vi "P-612 Stage Engine.vi"(0 "Unique Notifier Name":string, 11 "COM Port":string[](array[string])) -> ()   [LabVIEW 2016]
uses:
  Stages Controls/Stage Status.ctl
  Stages Controls/Stage XY Control.ctl
  Stages Controls/Stage Notifier Element.ctl
  Stages Controls/Stage Actions.ctl
panel:
  in  "XY Control":T1={"Left"=FALSE, "Right"=FALSE, "Up"=FALSE, "Down"=FALSE, "Home"=FALSE, "StageStep"=enum."1", "Y"=0.0, "X"=0.0}
  in  "ReInitialize":bool
  in  "Error":bool
  out "Status":T2
  in  "QUIT":bool
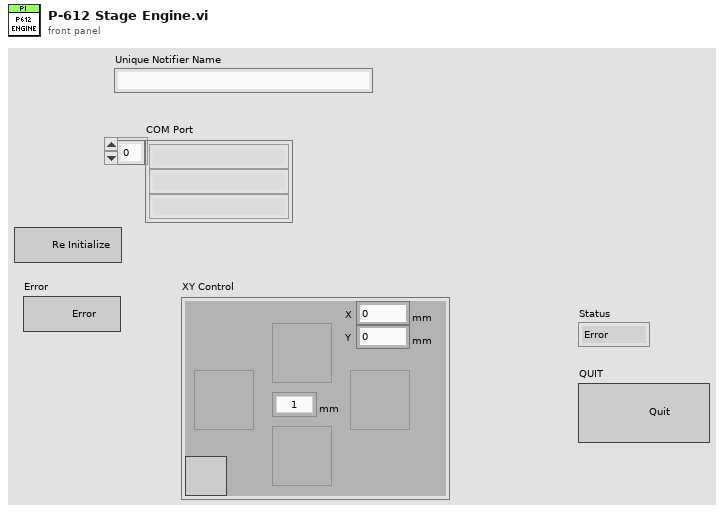
[diagram p1: front panel]
types:
  T1 = typedef "Stage XY Control.ctl" = cluster{"Left":bool, "Right":bool, "Up":bool, "Down":bool, "Home":bool, "StageStep":enum16{"0.01", "0.02", "0.05", "0.1", "0.5", "1", "2", "5", "10", "20", "50", "100", "500", "1000", "2000", "5000"}, "Y":dbl, "X":dbl}
  T2 = typedef "Stage Status.ctl" = enum16{"Error", "Abort", "Busy", "On Target"}
  T3 = typedef "Stage Actions.ctl" = enum16{"Get Position", "MVR", "MOVE", "HALT", "ONTARGET", "ERROR", "REFERENCE", "INIT", "VELOCITY", "STATUS", "EXIT", "HOME", "ZEROPOS", "NANOPOS", "ANALOG", "QUIT"}
  T4 = typedef "Stage Notifier Element.ctl" = cluster{"Action":T3, "Axis":bool[], "Setpoint":dbl[], "Velocity":dbl, "Cmd Recvd?":bool, "Position":dbl[], "Status":T2, "Misc":variant}
  T5 = cluster{"Left":bool, "Right":bool, "Up":bool, "Down":bool, "Home":bool, "StageStep":bool, "Y":bool, "X":bool}
  T6 = enum16{"0.01", "0.02", "0.05", "0.1", "0.5", "1", "2", "5", "10", "20", "50", "100", "500", "1000", "2000", "5000"}
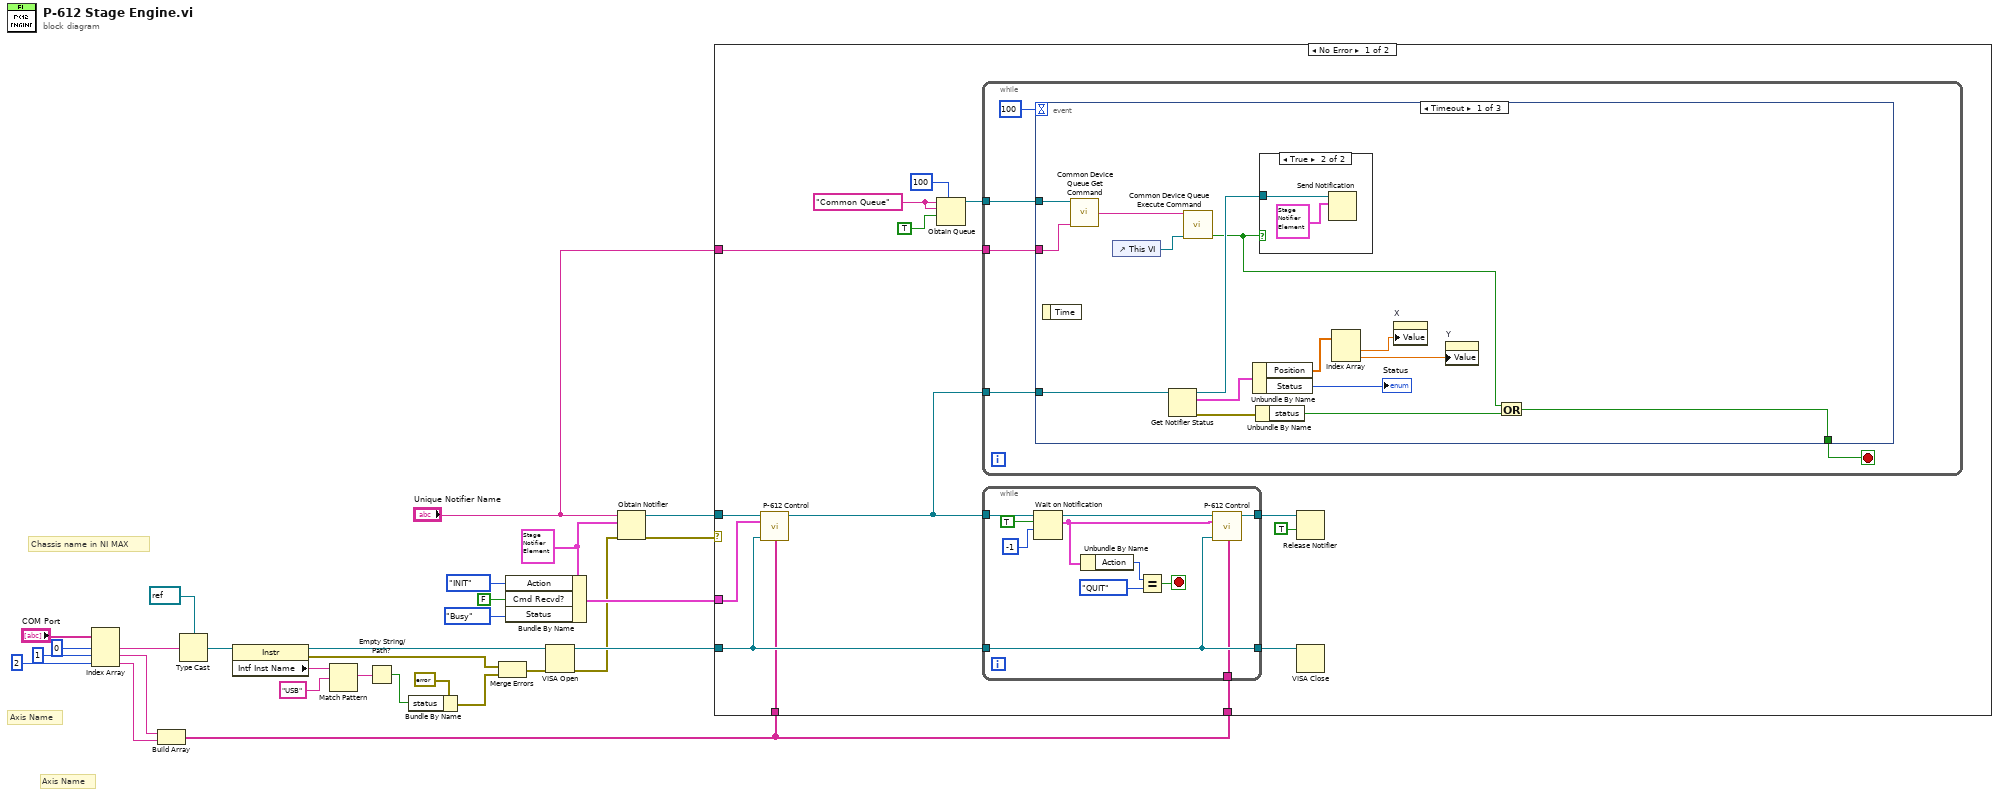
[diagram p0: block diagram]
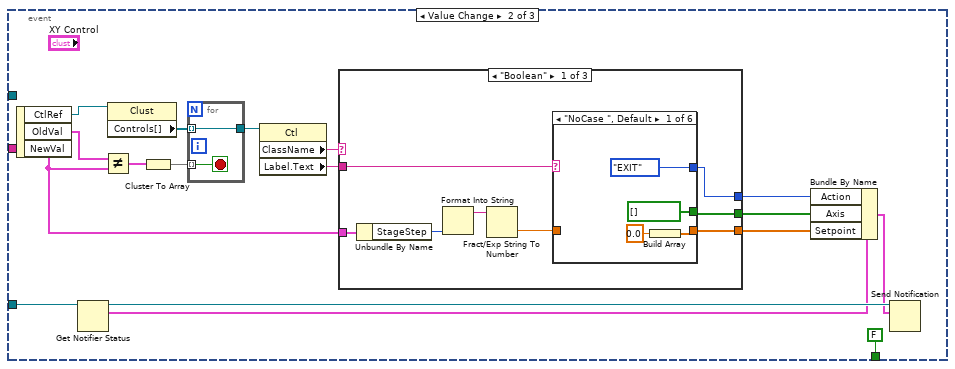
[diagram p3: hidden frame]
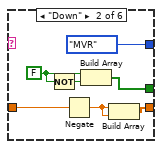
[diagram p4: hidden frame]
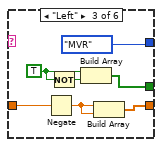
[diagram p5: hidden frame]
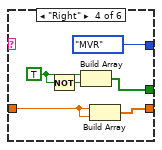
[diagram p6: hidden frame]
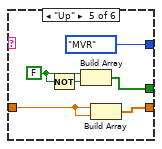
[diagram p7: hidden frame]
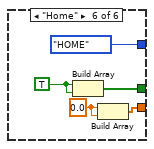
[diagram p8: hidden frame]
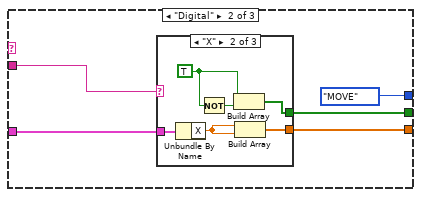
[diagram p9: hidden frame]
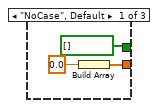
[diagram p10: hidden frame]
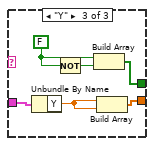
[diagram p11: hidden frame]
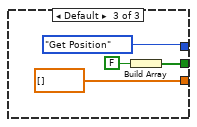
[diagram p12: hidden frame]
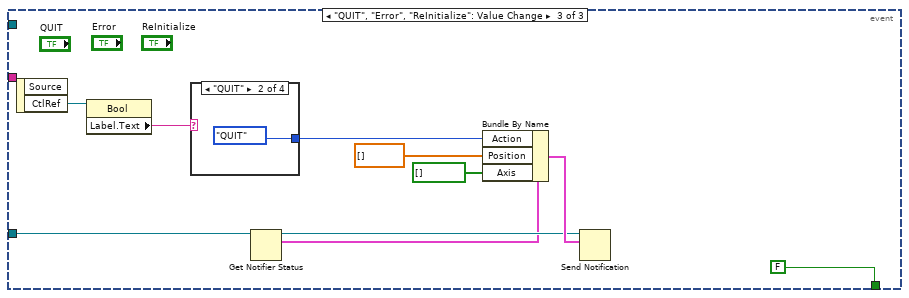
[diagram p13: hidden frame]
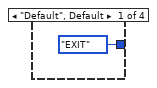
[diagram p14: hidden frame]
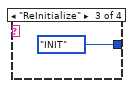
[diagram p15: hidden frame]
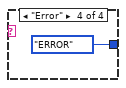
[diagram p16: hidden frame]
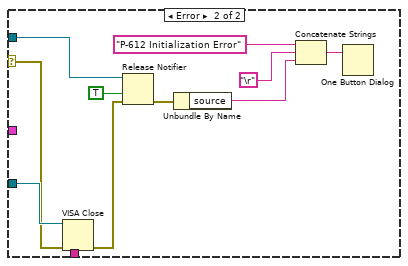
[diagram p17: hidden frame]
diagram:
  w15 = T4 {"Action"=enum."Get Position", "Axis"=[], "Setpoint"=[], "Velocity"=0.5, "Cmd Recvd?"=FALSE, "Position"=[], "Status"=enum."Abort", "Misc"=variant} ("Stage Status")
  # "Axis Name"
  # "Axis Name"
  # "Chassis name in NI MAX"
  n1 = Index Array(array="COM Port", index #1=0 ("index"), index #2=1 ("index"), index #3=2 ("index")) -> (element #1=w24:string, element #2=w3:string, element #3=w2:string)
  n2 = Build Array(w3, w2) -> (w1:string[])
  n3 = Type Cast(type=refnum<visa-resource-name> refnum ("reference out"), x=w24) -> (*(type *) &x=w22:refnum<visa-resource-name>)
  n4 = property class="Instr"(reference=w22) -> (reference out=w11:refnum<visa-resource-name>, error out=w19:errorcluster, "Intf Inst Name"=w27:string)  [unwired: 1 in]
  n5 = Match Pattern(string=w27, regular expression="USB") -> (match substring=w29:string)  [unwired: 1 in, 3 out]
  n6 = Empty String/Path?(string/path=w29) -> (empty?=w26:bool)
  n7 = Bundle By Name(cluster=errorcluster {"status"=FALSE, "code"=0, "source"=""} ("Error"), "status"=w26) -> (w20:errorcluster)
  n8 = Merge Errors(w19, w20) -> (w10:errorcluster)
  n9 = Bundle By Name(cluster=w15, "Action"=Stage_Actions."INIT", "Cmd Recvd?"=FALSE, "Status"=Stage_Status."Busy") -> (w12:T4)
  n10 = VISA Open(error in (no error)=w10, VISA resource name=w11) -> (VISA resource name=w9:refnum<visa-resource-name>, error out=w8:errorcluster)  [unwired: 3 in]
  n11 = Obtain Notifier(name (unnamed)="Unique Notifier Name", notification data type=w15, error in (no error)=w8) -> (notifier out=w13:refnum<notifier>, error out=w14:errorcluster)  [unwired: 1 in, 1 out]
  n12 = case shown="No Error" w14 {
    selector: w14 -> [_ w177]
    tunnel: w13 -> [w41 w179]
    tunnel: w12 -> [w40 _]
    tunnel: w9 -> [w39 w178]
    tunnel: "Unique Notifier Name" -> [w32 _]
    tunnel: w1 -> [w31 _]
    tunnel: w1 -> [w30 _]
    frame No Error {
      w35 = "Common Queue" ("Unique Notifier Name")
      n13 = call "P-612 Control.vi"("P-612 Notifier"=w41, "Stage Actions"=w40, "VISA In"=w39, "Axis Names"=w30) -> ("P-612 Notifier (Dup)"=w34:refnum<notifier>)  [unwired: 11 in]
      n14 = Obtain Queue(max queue size (-1, unlimited)=100, name (unnamed)=w35, element data type=w35, create if not found? (T)=TRUE) -> (queue out=w33:refnum<queue>)  [unwired: 1 in, 2 out]
      n15 = while {
        tunnel: w34 -> [w57]
        tunnel: w33 -> [w56]
        tunnel: w32 -> [w55]
        stop <- w58 stop-if-true
        n16 = event shown="[0] Timeout" {
          selector: _ -> [_ _ _]
          dyn-events: _ -> [_ _ _]
          timeout: 100 -> [_ _ _]
          tunnel: [w61 FALSE ("status") FALSE ("status")] -> w58
          tunnel: w57 -> [w68 w77 w163]
          tunnel: w56 -> [w65 _ _]
          tunnel: w55 -> [w64 _ _]
          event Timeout {
            n17 = event-data() -> ()  [unwired: 1 in, 1 out]
            n18 = call "Common Device Queue Get Command.vi"("Common Queue"=w65, "Notifier Name"=w64) -> ("Command"=w66:string)  [unwired: 12 in, 1 out]
            n19 = control-ref of="This VI"() -> (w67:refnum<vi>)
            n20 = Get Notifier Status(notifier=w68) -> (notifier out=w63:refnum<notifier>, current notification=w74:T4, error out=w72:errorcluster)  [unwired: 1 in, 2 out]
            n21 = call "Common Device Queue Execute Command.vi"("Common Command"=w66, "VI Refnum"=w67) -> ("Quit?"=w60:bool)  [unwired: 12 in, 1 out]
            n22 = Unbundle By Name(w74) -> ("Position"=w73:dbl[], "Status"=→"Status":T2)
            n23 = Unbundle By Name(w72) -> ("status"=w62:bool)
            n24 = case shown="True" w60 {
              tunnel: w63 -> [_ w76]
              frame False {
              }
              frame True {
                n25 = Send Notification(notification=T4 {"Action"=enum."QUIT", "Axis"=[], "Setpoint"=[], "Velocity"=0.5, "Cmd Recvd?"=FALSE, "Position"=[], "Status"=enum."Error", "Misc"=variant} ("Stage Status"), notifier=w76) -> ()  [unwired: 1 in, 2 out]
              }
            }
            n26 = Index Array(array=w73) -> (element #1=w70:dbl, element #2=w69:dbl)  [unwired: 2 in]
            n27 = property on="X" class="DigNum (strict)"("Value"=w70) -> ()  [unwired: 2 in, 2 out]
            n28 = property on="Y" class="DigNum (strict)"("Value"=w69) -> ()  [unwired: 2 in, 2 out]
            n29 = Or(x=w60, y=w62) -> (x .or. y?=w61:bool)
          }
          event Value Change {
            n30 = event-data() -> ("CtlRef"=w83:refnum<vi>, "OldVal"=w82:T1, "NewVal"=w81:T1)  [unwired: 1 in]
            n31 = Get Notifier Status(notifier=w77) -> (notifier out=w92:refnum<notifier>, current notification=w91:T4)  [unwired: 1 in, 3 out]
            n32 = Not Equal?(x=w82, y=w81) -> (x != y?=w89:T5)
            n33 = property class="Clust"(reference=w83) -> ("Controls[]"=w87:refnum<vi>[])  [unwired: 1 in, 2 out]
            n34 = Cluster To Array(cluster=w89) -> (array=w88:bool[])
            n35 = for {
              tunnel: w88 -> [w162] mode=indexing
              tunnel: [w161] -> w86
              tunnel: w87 -> [w161] mode=indexing
              stop <- w162 stop-if-true
            }
            n36 = property class="Ctl"(reference=w86) -> ("ClassName"=w85:string, "Label.Text"=w84:string)  [unwired: 1 in, 2 out]
            n37 = case shown="\"Boolean\"" w85 {
              tunnel: w81 -> [w101 w140 _]
              tunnel: w84 -> [w95 w141 _]
              tunnel: [w97 w139 dbl[] []] -> w80
              tunnel: [w98 w138 w159] -> w79
              tunnel: [w96 Stage_Actions."MOVE" ("Action") Stage_Actions."Get Position" ("Action")] -> w78
              frame "Boolean" {
                n38 = Unbundle By Name(w101) -> ("StageStep"=w99:T6)
                n39 = Format Into String(w99) -> (resulting string=w100:string)  [unwired: 3 in, 1 out]
                n40 = Fract/Exp String To Number(string=w100) -> (number=w94:dbl)  [unwired: 3 in, 1 out]
                n41 = case shown="\"NoCase \", Default" w95 {
                  tunnel: [w103 w108 w115 w122 w128 w134] -> w97
                  tunnel: [bool[] [] w109 w116 w123 w129 w136] -> w98
                  tunnel: w94 -> [_ w112 w119 w121 w127 _]
                  tunnel: [Stage_Actions."EXIT" ("Action") Stage_Actions."MVR" ("Action") Stage_Actions."MVR" ("Action") Stage_Actions."MVR" ("Action") Stage_Actions."MVR" ("Action") Stage_Actions."HOME" ("Action")] -> w96
                  frame "NoCase ", Default {
                    n42 = Build Array(0.0) -> (w103:dbl[])
                  }
                  frame "Down" {
                    w110 = FALSE
                    n43 = Not(x=w110) -> (.not. x?=w111:bool)
                    n44 = Negate(x=w112) -> (-x=w107:dbl)
                    n45 = Build Array(w110, w111) -> (w109:bool[])
                    n46 = Build Array(w107, w107) -> (w108:dbl[])
                  }
                  frame "Left" {
                    w117 = TRUE
                    n47 = Negate(x=w119) -> (-x=w114:dbl)
                    n48 = Not(x=w117) -> (.not. x?=w118:bool)
                    n49 = Build Array(w117, w118) -> (w116:bool[])
                    n50 = Build Array(w114, w114) -> (w115:dbl[])
                  }
                  frame "Right" {
                    w124 = TRUE
                    n51 = Not(x=w124) -> (.not. x?=w125:bool)
                    n52 = Build Array(w124, w125) -> (w123:bool[])
                    n53 = Build Array(w121, w121) -> (w122:dbl[])
                  }
                  frame "Up" {
                    w130 = FALSE
                    n54 = Not(x=w130) -> (.not. x?=w131:bool)
                    n55 = Build Array(w130, w131) -> (w129:bool[])
                    n56 = Build Array(w127, w127) -> (w128:dbl[])
                  }
                  frame "Home" {
                    w133 = 0.0
                    w135 = TRUE
                    n57 = Build Array(w135, w135) -> (w136:bool[])
                    n58 = Build Array(w133, w133) -> (w134:dbl[])
                  }
                }
              }
              frame "Digital" {
                n59 = case shown="\"X\"" w141 {
                  tunnel: [bool[] [] w149 w154] -> w138
                  tunnel: w140 -> [_ w148 w153]
                  tunnel: [w142 w147 w152] -> w139
                  frame "NoCase", Default {
                    n60 = Build Array(0.0 ("Y axis (mm)")) -> (w142:dbl[])
                  }
                  frame "X" {
                    w150 = TRUE
                    n61 = Unbundle By Name(w148) -> ("X"=w146:dbl)
                    n62 = Not(x=w150) -> (.not. x?=w145:bool)
                    n63 = Build Array(w150, w145) -> (w149:bool[])
                    n64 = Build Array(w146, w146) -> (w147:dbl[])
                  }
                  frame "Y" {
                    w156 = FALSE
                    n65 = Unbundle By Name(w153) -> ("Y"=w151:dbl)
                    n66 = Not(x=w156) -> (.not. x?=w155:bool)
                    n67 = Build Array(w156, w155) -> (w154:bool[])
                    n68 = Build Array(w151, w151) -> (w152:dbl[])
                  }
                }
              }
              frame Default {
                n69 = Build Array(FALSE) -> (w159:bool[])
              }
            }
            n70 = Bundle By Name(cluster=w91, "Action"=w78, "Axis"=w79, "Setpoint"=w80) -> (w90:T4)
            n71 = Send Notification(notification=w90, notifier=w92) -> ()  [unwired: 1 in, 2 out]
          }
          event "QUIT", "Error", "ReInitialize": Value Change {
            n72 = event-data() -> ("CtlRef"=w166:refnum<vi>)  [unwired: 1 in, 1 out]
            n73 = property class="Bool"(reference=w166) -> ("Label.Text"=w165:string)  [unwired: 1 in, 2 out]
            n74 = case shown="\"QUIT\"" w165 {
              tunnel: [Stage_Actions."EXIT" ("Action") Stage_Actions."QUIT" ("Action") Stage_Actions."INIT" ("Action") Stage_Actions."ERROR" ("Action")] -> w164
              frame "Default", Default {
              }
              frame "QUIT" {
              }
              frame "ReInitialize" {
              }
              frame "Error" {
              }
            }
            n75 = Get Notifier Status(notifier=w163) -> (notifier out=w168:refnum<notifier>, current notification=w167:T4)  [unwired: 1 in, 3 out]
            n76 = Bundle By Name(cluster=w167, "Action"=w164, "Position"=dbl[] [], "Axis"=bool[] []) -> (w169:T4)
            n77 = Send Notification(notification=w169, notifier=w168) -> ()  [unwired: 1 in, 2 out]
          }
        }
      }
      n78 = while {
        tunnel: [w47] -> w42
        tunnel: w34 -> [w49]
        tunnel: w39 -> [w46]
        tunnel: [w46] -> w38
        tunnel: w31 -> [w44]
        stop <- w54 stop-if-true
        n79 = Wait on Notification(notifier=w49, ignore previous (F)=TRUE, timeout in ms (-1)=-1) -> (notifier out=w48:refnum<notifier>, notification=w45:T4)  [unwired: 1 in, 2 out]
        n80 = Unbundle By Name(w45) -> ("Action"=w51:T3)
        n81 = Equal?(x=w51, y=Stage_Actions."QUIT") -> (x = y?=w54:bool)
        n82 = call "P-612 Control.vi"("P-612 Notifier"=w48, "Stage Actions"=w45, "VISA In"=w46, "Axis Names"=w44) -> ("P-612 Notifier (Dup)"=w47:refnum<notifier>)  [unwired: 11 in]
      }
      n83 = Release Notifier(notifier=w42, force destroy? (F)=TRUE) -> ()  [unwired: 1 in, 3 out]
      n84 = VISA Close(VISA resource name=w38) -> ()  [unwired: 1 in, 1 out]
    }
    frame Error {
      n85 = VISA Close(VISA resource name=w178, error in (no error)=w177) -> (error out=w180:errorcluster)
      n86 = Release Notifier(notifier=w179, force destroy? (F)=TRUE, error in (no error)=w180) -> (error out=w185:errorcluster)  [unwired: 2 out]
      n87 = Unbundle By Name(w185) -> ("source"=w182:string)
      n88 = Concatenate Strings("P-612 Initialization Error", "\r", w182) -> (w181:string)
      n89 = One Button Dialog(message=w181) -> ()  [unwired: 1 in, 1 out]
    }
  }
